vi "AlliGator Parameter Map Panel.vi"() -> ()   [LabVIEW 2021, in "AlliGator Parameter Map.lvlib"]
uses:
  AlliGator Parameter Map.lvlib
  AlliGator Parameter Map Control Refnums.ctl
  Globals, Variables, Constants/AlliGator Refnums List.ctl
  Utilities/Read-Write.ctl
  Settings/AlliGator Settings List.ctl
  Action Engine/AlliGator Q Element.ctl
  Action Engine/AlliGator Q Event.ctl
  Globals, Variables, Constants/AlliGator Variables List.ctl
  Palette/Image Palette Information.ctl
  Image/Image Display Palette Type.ctl
  Image/Image Display Event.ctl
  Image/Image Control Refnum.ctl
  <vilib>/Utility/miscctls.llb/LVPoint32TypeDef.ctl
  AlliGator Parameter Map Update Event Data.ctl
  GUI/AlliGator Image Mouse Up Event Data.ctl
  Image/Image ROI Descriptor.ctl
  Image/Image Contour Definition.ctl
  Image/Image Contour ID.ctl
  Image/Image ROI Type.ctl
  AlliGator Parameter Map Display Range Mouse Move Data.ctl
  Variant/Variant to Data/Variant to Boolean.vi
  Variant/Variant to Data/Variant to [String].vi
  Settings/AlliGator Settings+.lvlib
  Variant/Variant to Data/Variant to Data.lvlib
  Notebook/Notebook.lvlib
  Action Engine/AlliGator Action Engine.lvlib
  GUI/GUI.lvlib
  GUI/AlliGator GUI.lvlib
  Error/Error.lvlib
  Image/Image.lvlib
  Palette/Palette.lvlib
  Globals, Variables, Constants/AlliGator Globals, Variables & Constants.lvlib
  Python Plugins API/AlliGator Python Plugins.lvlib
  Phasor Plot/AlliGator Phasor Plot.lvlib
  Utilities/Utilities.lvlib
panel:
  in  "Map Parameter":u16(ring)
  in  "Parameter Map Set":u16(ring)
  in  "Pin Button":bool=TRUE
  in  "Overlay Parameter Map":bool caption="Overlay Decay Fit Parameter Map"
  in  "Parameter ROI Color":u32(colorbox)=6618880 caption="Phasor Plot ROI Color"
  in  "Refresh Parameter Map":bool caption="Refresh Phsor Plot"
  out "Parameter Map Display":T1(plugin-control)
  out "Parameter Map Value":dbl caption="Map Value" format="%#_5e"
  out "Parameter Map Y":i32 caption="Y"
  out "Parameter Map X":i32 caption="X"
  out "Min Parameter":dbl format="%#_5e"
  out "Max Parameter":dbl=1.0 format="%#_5e"
  in  "Parameter Map Color Scale":dbl(ramp)
  in  "Parameter Map Display Range":cluster{dbl, dbl}(slide)={0.0, 1.0} scale=9931.5..63525.26 scale format="%04_3g"
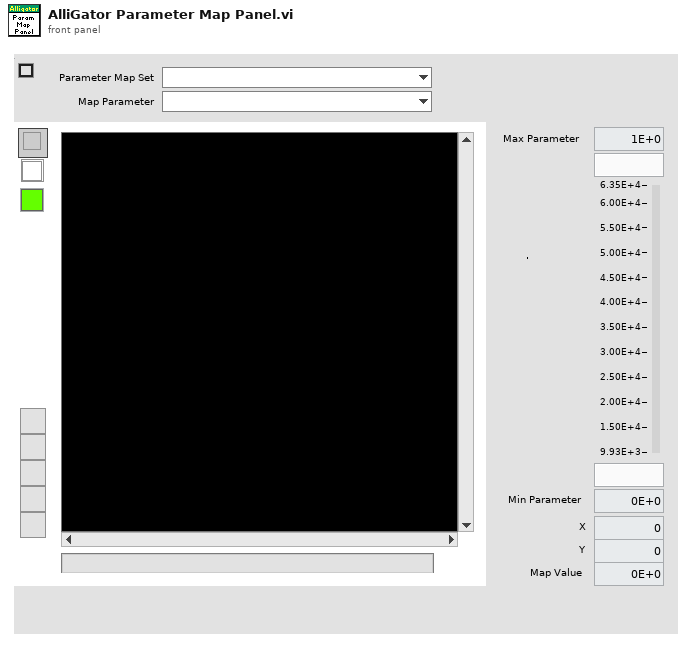
[diagram p1: front panel]
types:
  T1 = typedef "IMAQ Image.ctl" = refnum<image>
  T2 = typedef "Utilities.lvlib/Read-Write.ctl" = enum16{"Read", "Write"}
  T3 = typedef "AlliGator GUI.lvlib/AlliGator Refnums List.ctl" = enum16{"---------- AlliGator Control Refnums ----------", "AlliGator Tab Control Refnum", "Dataset Ctrl Refnums", "Image Histogram Ctrl Refnums", "Intensity Time Trace Ctrl Refnums", "Decay Graph Ctrl Refnums", "Decay Statistics Graph Ctrl Refnums", "Phasor Graph Ctrl Refnums", "Phasor Ratio Graph Ctrl Refnums", "Phasor Plot Ctrl Refnums", "Lifetime & Other Parameters Ctrl Refnums", "Decay Fit Parameter Map Ctrl Refnums", "Parameter Map Ctrl Refnums", "Other AlliGator Ctrl Refnums", "---------- AlliGator Menu Refnums ----------", "AlliGator Menu", "---------- IO Device ID ----------", "Mouse ID", "Keyboard ID"}
  T4 = typedef "AlliGator Parameter Map.lvlib/AlliGator Parameter Map Control Refnums.ctl" = cluster{"Parameter Map Color Scale":refnum<vi>, "Map Parameter":refnum<vi>, "Max Parameter":refnum<vi>, "Min Parameter":refnum<vi>, "Parameter Map Display":refnum<vi>, "Parameter Map Display Range":refnum<vi>, "Parameter Map Set":refnum<vi>, "Parameter Map X":refnum<vi>, "Parameter Map Y":refnum<vi>, "Parameter Map Value":refnum<vi>}
  T5 = cluster{"Event Registration Refnum":refnum<event-registration>, "Parameter Map Display Range Event":refnum<event-registration>, "Parameter Map Display Event":refnum<event-registration>}
  T6 = typedef "AlliGator Settings+.lvlib/AlliGator Settings List.ctl" = enum16{"GUI:Visible Settings Tab", "GUI:Last Run Version", "Source Image:Use Image Histogram for Contrast", "Source Image:Low Count Pixels Rejection Options", "Source Image:High Count Pixels Rejection Options", "Source Image:Use Image Brightness", "Source Image:Blend Overlay with Image Background", "Source Image:Use Fixed ROI Diameter", "Source Image:ROI Diameter", "Source Image:ROI Center Color", "Source Image:Peak Threshold", "Source Image:Intensity Threshold", "Source Image:Image Binning Options", "Source Image:Image Smoothing Options", "Source Image:Image Histogram Active", "Source Image:Invert Binary Mask", "Source Image:Hot Pixel Removal", "Source Image:Overlay Analyzed ROI Center", "Source Image:Auto-Adjust Contrast", "Source Image:Histogram Lower Percentile", "Source Image:Histogram Upper Percentile", "Source Image:Lock ROI with Maps", "Source Image:Save Source Image", "Source Image:Scale Bar Options", "Source Image:Image Resolution (Pixel Size)", "Source Image:Flatfield Correction", "Source Image:Show Dead Left Columns Correction", "Source Image:Dead Left Columns Correction", "Source Image:Image Pre-Processing Operations Order", "Source Image:Overlay ROI Median", "Source Image:Median Overlay Color", "Data Information:Gate Width", "Data Information:Nanotime Gate Separation", "Data Information:Macrotime Gate Separation", "Data Information:Gate Step", "Data Information:# Gates", "Data Information:Gate Image Exposure", "Data Information:Gate Image Integration", "Data Information:Gates to Skip", "Data Information:Gates to Keep", "Data Information:Define Gates to", "Data Information:Channel Name", "Data Information:Available Channel Names", "Data Information:Channel Arithmetic", "Data Information:Background File Subtraction", "Data Information:Background File", "Data Information:Background Scaling Factor", "Data Information:Background Pile-up Correction", "Data Information:Background Pixel Well Capacity", "Data Information:Laser Period", "Data Information:SYNC Period", "Data Information:Pile-up Correction", "Data Information:Pixel Well Capacity", "Data Information:Dataset Scaling Factor", "Fluorescence Decay_Decay Pre-Processing:Reverse Gates", "Fluorescence Decay_Decay Pre-Processing:Verbose Decay Pre-Processing", "Fluorescence Decay_Decay Pre-Processing:Use Decay Pre-Processing", "Fluorescence Decay_Decay Pre-Processing:Background Subtraction", "Fluorescence Decay_Decay Pre-Processing:Background Definition Range", "Fluorescence Decay_Decay Pre-Processing:Baseline Subtraction Method", "Fluorescence Decay_Decay Pre-Processing:Decay Pre-Processing Operations Order", "Fluorescence Decay_Decay Pre-Processing:Smoothing Parameter", "Fluorescence Decay_Decay Pre-Processing:Shift Decay", "Fluorescence Decay_Decay Pre-Processing:Decay Shift Parameters", "Fluorescence Decay_Decay Pre-Processing:Fold Decay", "Fluorescence Decay_Decay Pre-Processing:# Folds", "Fluorescence Decay_Decay Pre-Processing:1-Normalize Decay", "Fluorescence Decay_Decay Pre-Processing:[0-1]-Normalize Decay", "Fluorescence Decay_Decay Pre-Processing:Smoothen Decay", "Fluorescence Decay_Decay Pre-Processing:Extrapolate Decay", "Fluorescence Decay_Decay Pre-Processing:Use Periodicity", "Fluorescence Decay_Decay Pre-Processing:Use Cursors", "Fluorescence Decay_Decay Pre-Processing:Tail Fraction", "Fluorescence Decay_Decay Pre-Processing:Head Fraction", "Fluorescence Decay_Decay Pre-Processing:Additional Points", "Fluorescence Decay_Decay Pre-Processing:Straighten Decay", "Fluorescence Decay_Decay Pre-Processing:Constant Background", "Fluorescence Decay_Decay Pre-Processing:Pixel-Normalize Decay", "Fluorescence Decay_Advanced Analysis:Extract IRF instead of Decay", "Fluorescence Decay_Advanced Analysis:IRF Extraction Options", "Fluorescence Decay_Advanced Analysis:IRF Optimization Options", "Fluorescence Decay_Advanced Analysis:Square Pulse Options", "Fluorescence Decay_Advanced Analysis:IRF Order", "Fluorescence Decay_Advanced Analysis:IRF Time Constants", "Fluorescence Decay_Advanced Analysis:Wavelet Analysis Options", "Fluorescence Decay_Advanced Analysis:Average Lifetime Options", "Fluorescence Decay_Fit Options:Fit Options", "Fluorescence Decay_Fit Options:Use Legacy Fitting Approach", "Fluorescence Decay_Fit Options:Use Data Information Laser Period", "Fluorescence Decay_Fit Parameters:Displayed Fit Parameters", "Fluorescence Decay_Fit Parameters:Fit Parameter Constraints", "Fluorescence Decay_Fit Parameters:Export Tabulated Results", "Fluorescence Decay_Fit Parameters:MLE Baseline Offset Type", "Fluorescence Decay_Fit Parameters:MLE Baseline Offset", "Fluorescence Decay_Fit Parameters:Guess Parameter Names", "Fluorescence Decay_Fit Parameters:Guess Parameter Values", "Fluorescence Decay_Fit Parameters:Guess Parameters Options", "Fluorescence Decay_Fit Parameters:Optimal Offset Selection Criterion", "Fluorescence Decay_Styles:Show Last Decay Only", "Fluorescence Decay_Styles:Decay Graph Color Array", "Fluorescence Decay:Decay Graph Active", "Fluorescence Decay Statistics:Min Peak Value", "Fluorescence Decay Statistics:Reject Low Decay Peak Pixels", "Fluorescence Decay Statistics:Reject High Decay Peak Pixels", "Fluorescence Decay Statistics:Max Peak Value", "Time Traces:Use File Timestamp", "Time Traces:Time Step", "Time Traces:Use Intensity Correction File", "Time Traces:Intensity Correction File", "Phasor Plot:Phasor Plot Smoothing Options", "Phasor Plot:Phasor Plot Size", "Phasor Plot:Phasor Plot Graphics Options", "Phasor Plot:Cumulative Phasor Plot", "Phasor Plot:Use Phasor Brightness", "Phasor Plot:Blend Overlay with Phasor Background", "Phasor Plot:Save Phasor Plot", "Phasor Plot:Show References", "Phasor Plot:Phasor Ratio Decay Range", "Phasor Plot:Exponential Fading", "Phasor Plot:Phasor Ratio Reference Colors", "Phasor Plot:Reference Radius", "Phasor Plot:Show Color Map Vertices", "Phasor Plot:Phasor Plot Active", "Phasor Plot:Phasor Ratio Color Map Type", "Phasor Plot:Phasor Ratio Color Map", "Phasor Plot:Phasor Ratio Display Range", "Phasor Plot:Selected Image ROI(s)", "Phasor Plot:All Image ROIs", "Phasor Plot:Selected Phasor Plot ROI(s)", "Phasor Plot:All Phasor Plot ROIs", "Phasor Plot:Phasor Ratio Color-Coded Quantity", "Phasor Plot:Store Phasor Harmonics", "Phasor Plot:Draw Reference Segment", "Phasor Plot:User-Defined Quantity", "Phasor Plot:Color Scale High Color", "Phasor Plot:Color Scale Low Color", "Phasor Plot:Intensity-weighted Phasor Plot", "Phasor Graph:Phasor Frequency", "Phasor Graph:Phasor Ratio Type", "Phasor Graph:Pixel-level Phasor Computation", "Phasor Graph:Save Phasor Graph", "Phasor Graph:Phasor Graph Active", "Phasor Graph:Phasor SDV Options", "Phasor Graph:Intensity-weighted Phasor Graph", "Phasor Graph:Define Shortest Lifetime as", "Phasor Calibration:Use Backup Calibration if needed", "Phasor Calibration:Backup Calibration Type", "Phasor Calibration:Calibration Type", "Phasor Calibration:Calibration Lifetime", "Phasor Calibration:Calibration Map Algorithm", "Single-Exponential Phasor Locus (SEPL):Gate Parameters", "Single-Exponential Phasor Locus (SEPL):User-defined Gate", "Single-Exponential Phasor Locus (SEPL):User-defined IRF", "Single-Exponential Phasor Locus (SEPL):Phasor Parameters", "Single-Exponential Phasor Locus (SEPL):Decay & IRF Parameters", "Single-Exponential Phasor Locus (SEPL):Display Parameters", "Lifetime Analysis:Decay Analysis Parameters", "Lifetime Analysis:Lifetime Map Active", "Plugins:Python Settings", "Miscellaneous:Verbose Mode", "Miscellaneous:Beep after Script", "Miscellaneous:Saved Image File Format", "Miscellaneous:Exported Gate Image Settings", "Miscellaneous:Include Loading in Timing", "Miscellaneous:Verbose Settings Mode", "Miscellaneous:Histogram Options", "Miscellaneous:Beep on Error", "Miscellaneous:# Logical Processors Used", "Miscellaneous:ROI Description Max Characters", "Miscellaneous:Verbose Error Mode", "Miscellaneous:Transparent Mask Color"}
  T7 = typedef "AlliGator Action Engine.lvlib/AlliGator Q Element.ctl" = cluster{"AlliGator Q Event":T8, "Data":variant}
  T8 = typedef "AlliGator Action Engine.lvlib/AlliGator Q Event.ctl" = enum16{"---- Files ----", "Files:Set Batch Export Files To Save", "Files:Set Dataset Loading & Pre-processing Options", "Files:Check #Frames in Dataset", "Files:Increment Frame Index", "Files:Open Mask Image", "Files:Open White Light Image", "Files:Open Single Dataset", "Files:New Folder of Folders Selected", "Files:Load File (all Types)_Scriptable", "Files:Move Flattened Series to Folders Series", "Files:Select Folder", "Files:Load FLI Dataset", "Files:Load Swiss SPAD 1 Dataset", "Files:Load Swiss SPAD 2 Dataset", "Files:Load .sdt FLI Dataset", "Files:Load .ptu FLI Dataset", "Files:Load .bin FLI Dataset", "Files:Load Single Gate Image Folder", "Files:Load I/m/phi Dataset (deprecated)", "Files:Load Single Image", "Files:Subtract Background File", "Files:Export FLI Dataset", "Files:Load HDF5 FLI Dataset", "Files:Set Destination File Path", "Files:Save Mask Image", "Files:Batch Conversion", "Files:New Folder Selected", "Files:Close FLI Dataset", "Files:Close FLI Dataset Series", "Files:Close White Light Image", "Files:Close Mask Image", "---- FLI Dataset ----", "FLI Dataset:Channel Arithmetic", "FLI Dataset:Export Average Lifetime Map as ASCII", "FLI Dataset:Export User-Defined Quantity Map as ASCII", "FLI Dataset:Python Function FLI Dataset Event", "FLI Dataset:ROI Analysis", "FLI Dataset:Tilted Logistic Square Gated IRF Characteristics Map", "FLI Dataset:Logistic Square Gated IRF Characteristics Map", "FLI Dataset:Square Gated IRF Characteristics Map", "FLI Dataset:Multi-ROI Single-Pixel Phasor Analysis", "FLI Dataset:Multi-ROI Single-Pixel NLSF Analysis", "FLI Dataset:All ROIs IRF Extraction", "FLI Dataset:All ROIs Decay Fit Non-Interactive (Fast + Individual IRF)", "FLI Dataset:All ROIs Phasor Analysis", "FLI Dataset:All ROIs Decay Fit", "FLI Dataset:Fluorescence Decay Statistics", "FLI Dataset:Update Decay Statistics Graph", "FLI Dataset:Get Decay from ROI", "FLI Dataset:All ROIs Average Lifetimes", "FLI Dataset:Save/Load Local IRFs", "FLI Dataset:Clear Local IRFs", "FLI Dataset:Phasor Calibration Maps (# Gates Series) Script", "FLI Dataset:Calibrated Phasor Map Series", "---- FLI Dataset Series ----", "FLI Dataset Series:Sum All Datasets in Series", "FLI Dataset Series:Add Dataset to Accumulated Dataset", "FLI Dataset Series:Display Accumulated Dataset", "FLI Dataset Series:Clear Dataset Series Sum", "FLI Dataset Series:Time-Series Analysis (NLSF)", "FLI Dataset Series:Time-Series Analysis (Phasor)", "---- Image ----", "Image:Update Image Profile Plots", "Image:Image Histogram Cursor Move", "Image:Image Histogram", "Image:Image Contrast", "Image:Set Image Histogram Cursor Move Flag", "Image:Clear Image Overlay", "Image:Use ROI as Search Area", "Image:Set ROI Diameter", "Image:Save Image Data as TIFF", "Image:Save Displayed Image with Overlay", "Image:Save Image Overlay Only", "Image:Save Image as Hot Pixel Mask", "Image:Change Source Image Color Palette", "Image:Copy Image to Clipboard", "Image:Source Image ROI Selection", "Image:Delete All ROIs", "Image:Delete All Unselected ROIs", "Image:Delete ROI", "Image:Merge All ROIs", "Image:Store ROI", "Image:Source Image ROI Storage", "Image:Export ROI Description to Notebook", "Image:Save ROI", "Image:Load ROI", "Image:Paste ROI Definition", "Image:Clear ROI", "Image:Identify ROIs in Mask Image", "Image:Create Complementary ROI", "Image:Create Contour ROI", "Image:Create ROI(s) from Pixels with Peak above Min_Scriptable", "Image:Create ROI(s) from Pixels with Intensity above Min_Scriptable", "Image:Compute ROI Statistics", "Image:Delete ROI(s) based on ROI Characteristics", "Image:Create ROI Grid", "Image:ROI to Individual Pixel ROIs", "Image:Python Function Source Image Event", "Image:Show Phasor Calibration Map ROI Centers", "Image:Convert ROI to Mask Image", "Image:Mouse Move", "Image:Mouse Up", "Image:Set Source Image Mouse Move Flag", "Image:Add Scale Bar Overlay", "Image:Delete Existing ROIs Option", "Image:Overlay ROI Median", "Image:Check Current ROI", "Image:Update True Pixel Value", "Image:Use ROI", "---- Decay ----", "Decay:Clear IRF/Reference Plot", "Decay:Add Decay to Graph", "Decay:Smoothen Plot", "Decay:Smoothen Plot Tail", "Decay:Average Selected Plots", "Decay:Extract IRF", "Decay:Optimal IRF Extraction", "Decay:Threshold IRF", "Decay:Fit to Model IRF", "Decay:Fit IRF to Square Gate", "Decay:Fit IRF to Logistic Square Gate", "Decay:Fit IRF to Tilted Logistic Square Gate", "Decay:Create Bounding Cursors Set", "Decay:Export Bounding Cursors Definition to Notebook", "Decay:Denoise Plot", "Decay:Compute Cumulative Function", "Decay:Use as Reference Decay", "Decay:Show Reference Decay/IRF", "Decay:Extrapolate Decay", "Decay:Create Head & Tail Bounding Cursors", "Decay:Store Cursor-defined Head & Tail Fractions", "Decay:Rebin Plot", "Decay:1-Normalize Decay", "Decay:[0-1]-Normalize Plot", "Decay:Straighten Decay", "Decay:Shift Decay", "Decay:Fold Decay", "Decay:Fit Decay", "Decay:Global Fit of Selected Decays", "Decay:Post Global Fit Script", "Decay:Add Global Fit Parameters to Graph", "Decay:Add Decay Parameter(s) to Plot (Graph)", "Decay:Export Decay to Phasor Graph", "Decay:Compute Average Lifetime", "Decay:Plot Convolution", "Decay:Graph Tip Strip Update", "---- Decay Statistics ----", "Decay Statistics:Tip Strip Update", "---- Intensity Time Trace ----", "Intensity Time Trace:Use File Timestamp", "Intensity Time Trace:Load Intensity Corrections File", "Intensity Time Trace:Clear Intensity Corrections File", "Intensity Time Trace:Tip Strip Update", "---- Phasor Plot ----", "Phasor Plot:Build Phasor Plot", "Phasor Plot:Change Phasor Plot Color Palette", "Phasor Plot:Adjust Phasor Plot Display Range", "Phasor Plot:Highlight Image ROI in Phasor Plot", "Phasor Plot:Save Phasor Plot Image with Overlay", "Phasor Plot:Export Complex Phasor Map", "Phasor Plot:Export Phasor Ratio Map", "Phasor Plot:Export Average Lifetime Map", "Phasor Plot:Compute Phase Lifetime Histogram", "Phasor Plot:Compute Phasor Ratio Histogram", "Phasor Plot:Compute Phase Lifetime vs Intensity Scatter Plot", "Phasor Plot:Weber 2-Component Decomposition", "Phasor Plot:Update Phasor Color Map Vertices", "Phasor Plot:Clear Phasor Overlay", "Phasor Plot:Use Segment Extremities as References", "Phasor Plot:Use UC/Segment Intersections as References", "Phasor Plot:Use UC/Principal Axis Intersections as References", "Phasor Plot:Use UC/Linear Fit Intersections as References", "Phasor Plot:Update Phasor Plot Reference", "Phasor Plot:Show Local Phasor Info in Phasor Plot", "Phasor Plot:Update Phasor Plot State", "Phasor Plot:Phasor Plot ROI Storage", "Phasor Plot:Phasor Plot ROI Selection", "Phasor Plot:Python Function Phasor Plot Event", "Phasor Plot:Overlay Phasor ROI, Ratio or Map in Source Image", "Phasor Plot:Compute Decay of Selected Phasors", "Phasor Plot:Phasor at Image Pixel", "Phasor Plot:Mouse Move", "Phasor Plot:Mouse Up", "Phasor Plot:Display Range Mouse Move", "Phasor Plot:Set Mouse Move Flag", "Phasor Plot:Update True Phasor Plot Value", "---- Phasor Graph ----", "Phasor Graph:Get Phasor Value", "Phasor Graph:Create New Phasor Plot Dialog", "Phasor Graph:Update Last Phasor Value", "Phasor Graph:Update Phasor (m, phi)", "Phasor Graph:Remove Single Phasor from Plot", "Phasor Graph:Add Single Phasor to Plot", "Phasor Graph:Remove Phasor Plot", "Phasor Graph:Remove Selected Phasor Plots", "Phasor Graph:Clear Phasor Data", "Phasor Graph:Clear Phasor Graph", "Phasor Graph:Cursor Move", "Phasor Graph:Draw Cursor Connecting Line", "Phasor Graph:Clear Cursor Connecting Line", "Phasor Graph:Find UC Intersection", "Phasor Graph:Use UC/Cursor-Defined Line Intersections", "Phasor Graph:Use Selected Plots Fitted Line/UC Intersections", "Phasor Graph:Use Selected Plots Principal Axis/UC Intersections", "Phasor Graph:Show Single Phasor", "Phasor Graph:Save Single Phasor Plot", "Phasor Graph:Save All Phasor Plots", "Phasor Graph:Load Phasor Plot(s)", "Phasor Graph:Phasor Multiplication", "Phasor Graph:Compute Average Phasor", "Phasor Graph:Compute Multiple Average Phasors (Selected Plots)", "Phasor Graph:Export Single Phasor Plot Phase Lifetimes", "Phasor Graph:Parameter 2 vs Parameter 1 Scatter Plot", "Phasor Graph:Use Cursor n Location", "Phasor Graph:Set Reference n to Current Phase Lifetime Value", "Phasor Graph:Set Reference n to Lifetime Value", "Phasor Graph:Set Cursor n Location", "Phasor Graph:Save Phasor Graph Image", "Phasor Graph:Update SEPL Plot", "Phasor Graph:Export Single Phasor Plot Data", "Phasor Graph:Export Selected Phasor Plots Data", "Phasor Graph:Python Function Phasor Graph Event", "Phasor Graph:Tip Strip Update", "---- Calibration ----", "Calibration:Set Calibration Type", "Calibration:Load/Save Phasor Calibration", "Calibration:Load/Save Phasor Calibration Series", "Calibration:Load/Save Phasor Calibration Map", "Calibration:Use as Calibration", "Calibration:Compute Optimal Calibration from Phasor References", "Calibration:Clear Phasor Calibration", "Calibration:Single Phasor Calibration Information", "Calibration:Use as Calibration Series", "Calibration:Use as Calibration Map", "Calibration:Clear Calibration Series", "Calibration:Phasor Calibration Series Information", "Calibration:Clear Calibration Map", "Calibration:Phasor Calibration Map Information", "Calibration:Apply Phasor Calibration", "Calibration:Update Single Plot Calibration", "Calibration:Update Multiple Plots Calibration", "Calibration:Clear Single Plot Calibration", "Calibration:Clear All Plots Calibrations", "Calibration:Clear Plot(s) Calibration(s)?", "---- Phasor Ratio ----", "Phasor Ratio:Clear Reference n", "Phasor Ratio:Toggle Selected Plot(s)  Lock to Reference 1", "Phasor Ratio:Use as Reference n", "Phasor Ratio:Send Reference n to Notebook", "Phasor Ratio:Toggle Selected Plot(s)  Lock to Reference 2", "Phasor Ratio:Compute Phasor Ratio at Mouse Location", "Phasor Ratio:Compute Phasor Plot's Average Phasor Ratio", "Phasor Ratio:Compute Time-Series Phasor Ratios", "Phasor Ratio:Fit Line to Phasor Ratio Plot", "Phasor Ratio:Save References", "Phasor Ratio:Load References", "Phasor Ratio:Update Phasor Reference 1", "Phasor Ratio:Update Phasor Reference 2", "Phasor Ratio:Move Cursor n to Reference n", "Phasor Ratio:Use as Phasor Reference 1 Lifetime", "Phasor Ratio:Use as Phasor Reference 2 Lifetime", "Phasor Ratio:Export Phasor Ratio Map as ASCII", "Phasor Ratio:Tip Strip Update", "---- Lifetime & Other Parameters Graph ----", "Lifetime:Compute Sliced Mean, SDV and CV Plots", "Lifetime:Plot Decay Shifts", "Lifetime:Plot Histogram", "---- Decay Fit Parameter Map ----", "Decay Fit Parameter Map:Export ROI NLSF Data as ASCII", "Decay Fit Parameter Map:Set Decay Fit Parameter Map Selection", "Decay Fit Parameter Map:Build Decay Fit Parameter Map", "Decay Fit Parameter Map:Change Decay Fit Parameter Map Color Palette", "Decay Fit Parameter Map:Export Decay Fit Parameter Map Data as ASCII", "Decay Fit Parameter Map:Export All Decay Fit Parameter Maps Data as ASCII", "Decay Fit Parameter Map:Selected Parameter Scatterplot", "Decay Fit Parameter Map:Parameter 2 vs Parameter 1 Scatterplot", "Decay Fit Parameter Map:Save Decay Fit Parameter Map Image", "Decay Fit Parameter Map:Save-Load IRFs & Fit Data", "Decay Fit Parameter Map:Update Local Decay Plots", "Decay Fit Parameter Map:Python Function Decay Fit Parameters Map Event", "Decay Fit Parameter Map:Overlay Decay Fit Parameter Map in Source Image", "Decay Fit Parameter Map:Selected Parameter vs Intensity Scatterplot", "Decay Fit Parameter Map:Mouse Up", "Decay Fit Parameter Map:Mouse Move", "Decay Fit Parameter Map:Display Range Mouse Move", "Decay Fit Parameter Map:Change Map Resolution", "Decay Fit Parameter Map:Variance Significance Maps", "Decay Fit Parameter Map:Fit Result Constraints Window", "Decay Fit Parameter Map:Use ROI", "---- Parameter Map ----", "Parameter Map:Export ROI Parameters Data as ASCII", "Parameter Map:Add Parameter Map Set", "Parameter Map:Delete Parameter Map Set", "Parameter Map:Update Parameter List", "Parameter Map:Build Parameter Map", "Parameter Map:Change Parameter Map Color Palette", "Parameter Map:Export Parameter Map Data as ASCII", "Parameter Map:Export All Parameter Maps Data as ASCII", "Parameter Map:Selected Parameter Scatterplot", "Parameter Map:Parameter 2 vs Parameter 1 Scatterplot", "Parameter Map:Selected Parameter vs Intensity Scatterplot", "Parameter Map:Save Parameter Map Image", "Parameter Map:Save-Load IRFs & Parameter Maps (TODO)", "Parameter Map:Set Parameter Map Selection", "Parameter Map:Python Function Parameter Map Event", "Parameter Map:Overlay Parameter Map in Source Image", "Parameter Map:Update Local Decay Plots", "Parameter Map:Mouse Up", "Parameter Map:Mouse Move", "Parameter Map:Display Range Mouse Move", "Parameter Map:Use ROI", "---- Generic Graph ----", "Generic Graph:Generic XY Graph Event", "Generic Graph:Python Function XY Graph Event", "Generic Graph:New Plot", "Generic Graph:Save Plot", "Generic Graph:XY Plot Histogram", "Generic Graph:Set XY Graph Plot Name", "Generic Graph:Set Last Cursor Style", "Generic Graph:Tip Strip Update", "---- GUI ----", "GUI:Start Script", "GUI:Type of Displayed Image Changed", "GUI:Gate Image Slide Changed", "GUI:Show Busy Icon", "GUI:Show Busy Icon & Abort Button", "GUI:Hide Busy Icon", "GUI:Hide Busy Icon & Abort Button", "GUI:Abort", "GUI:End Script", "GUI:Start Timing", "GUI:End Timing", "GUI:Set State Indicator", "GUI:Send Parameters JSON Strings to Clipboard", "GUI:Set Gate Step", "GUI:Idle", "GUI:Initialization", "GUI:Quit", "GUI:Increment Dataset Index", "GUI:Set Dataset Index to -1", "GUI:Time Series Slider Moved", "GUI:Time Series Slider Changed", "GUI:Toggle Playback or Loop", "GUI:Playback Script", "GUI:Set Phasor Frequency", "GUI:Open Window", "GUI:Start Test Script", "GUI:End Test Script", "GUI:Set Verbose Mode", "GUI:Set Verbose Settings Mode", "GUI:Initialize Python Session", "DEBUG"}
  T9 = typedef "Palette.lvlib/Image Palette Information.ctl" = cluster{"Palette Name [# Colors,int?,inv?]":string, "Palette Type":T10, "Palette Colors":u32[], "Interpolate?":bool}
  T10 = typedef "Image.lvlib/Image Display Palette Type.ctl" = u32
  T11 = typedef "AlliGator Globals, Variables & Constants.lvlib/AlliGator Variables List.ctl" = enum16{"---- GUI ----", "GUI:Initialization Status", "GUI:State Indicators Refnum", "GUI:Original AlliGator Menu Items", "GUI:Current Action Loop State", "GUI:Script in progress", "GUI:Playback", "GUI:Loop Playback", "GUI:Search ROI Used", "GUI:Search ROI", "Image Histogram Max Legend Size", "Decay Graph Max Legend Size", "Intensity Graph Max Legend Size", "Decay Statistics Graph Max Legend Size", "Phasor Graph Max Legend Size", "Phasor Ratio Graph Max Legend Size", "Lifetime Graph Max Legend Size", "---- Files ----", "Files:Export Dataset Frames as Individual Files", "Files:Show Batch Export Help Balloons", "Files:Frames in Dataset", "Files:ptu File Frame Start Indices", "Files:Current Frame in Dataset", "Files:Current Frame Timestamp", "Files:Dataset Loaded", "Files:Dataset Metadata", "Files:Dataset Channel", "Files:Dataset Data Description", "Files:Background Dataset Metadata", "Files:Background Dataset Channel", "Files:Background Dataset Data Description", "Files:Background File Subtraction", "Files:Background File Path", "Files:Background File Pile-up Correction", "Files:Background File Pixel Well Capacity", "Files:Background File Scaling Factor", "Files:Current Dataset Load Settings", "Files:Dataset Path", "Files:ICCD-specific Information", "Files:Macrotime Gate Separation", "------ Python Plugins ------", "Python Plugins:Information", "Python Plugins:Python Session", "Python Plugins:Valid Python Session?", "---- Source Image ----", "Source Image:ROIs", "Source Image:Current ROI", "Source Image:ROI Event Refnum", "X_Source Image:Display Range", "X_Source Image:Palette Information", "X_Source Image:Type of Displayed Image", "X_Time Gate Slider", "Source Image:Palette List", "Source Image:Scale", "Source Image:ROI Overlay Color", "Source Image:Overlay to Erase", "Source Image:Is Displayed Image Accumulated", "Source Image:White Light Image Modified", "Source Image:Mask Image Modified", "---- Image Profile Window ----", "Image Profile:Window Event Refnum", "Image Profile:IntensityType", "Image Profile:Intensity Average Type", "Image Profile:Intensity-weighted SDV", "Image Profile:Box Profile Type", "Image Profile:Window Open", "Image Profile:Plotted Fit Parameter", "------ Phasor Graph -------", "Phasor Graph:Show Line", "---- Phasor Plot ---", "Phasor Plot:Parameters Changed", "Phasor Plot:FLI Dataset Modified since last Calculation", "Phasor Harmonics Data", "Selected Phasor Harmonics", "Phasor Harmonic Manager Event Refnum", "Phasor Plot:ROIs", "Phasor Plot:Current ROI", "Phasor Plot:ROI Event Refnum", "Phasor Plot:Image Reference Points", "Phasor Plot:Computed", "Phasor Plot:Palette Information", "Phasor Plot:Palette List", "Phasor Plot:Phasor Ratio Palette Information", "Phasor Plot:Phasor Ratio Palette List", "Phasor Plot:Image Scale", "Phasor Plot:Image Overlay to Erase", "Phasor Plot:Image Elements to Update", "Phasor Plot:Current Calculation Parameters", "Phasor Plot:Current Calibration Options", "Phasor Plot:Reset Cumulated Phasor Plot", "Phasor Plot:Reference 1", "Phasor Plot:Lifetime Reference 1", "Phasor Plot:Reference 1 Frequency", "Phasor Plot:Reference 2", "Phasor Plot:Lifetime Reference 2", "Phasor Plot:Reference 2 Frequency", "---- Decay Analysis ----", "Number of Selected Decays to Fit", "LS Fit Results", "LAR Fit Results", "BS Fit Results", "Last Decay Max - Min", "Best Fit Parameters", "Best Fit Parameter Names", "Actual Size X", "Actual Size Y", "Binning X", "Binning Y", "Actual # Gates", "Dataset Number", "Gates to...", "Gates Skipped", "Gates to keep", "Gate Step", "Gate Separation", "Reversed Gates", "Pile-up Correction", "Pixel Well Capacity", "Background Subtracted", "Background Subtraction Method", "Background Definition Range", "Background File (deprecated)", "Number of Dataset Accumulated", "Array of Accumulated Dataset Paths", "Do Averaged Datasets", "Destination File Path", "Process Plot Target", "Use 1/D as Phasor Frequency", "---- Decay Fit Parameter Map -----", "Decay Fit Parameter Map:Palette Information", "Decay Fit Parameter Map:Palette List", "Decay Fit Parameter Map:X Resolution", "Decay Fit Parameter Map:Y Resolution", "Decay Fit Parameter Map:Use Decay Fit Result Constraints", "Decay Fit Parameter Map:Decay Fit Result Constraints", "Decay Fit Parameter Map:Decay Fit Result Constraints Applied", "---- Parameter Map ----", "Parameter Map:Palette Information", "Parameter Map:Palette List", "------- Local Decay Window ---------", "Local Decay Graph Window:Event Refnum", "Local Decay Graph Window:Use normalized IRF for convolution", "----- Miscellaneous ----", "Misc:Skippable Dialog Windows Status"}
  T12 = enum16{"0", "1", "2", "3", "4", "5", "6", "7", "8", "9", "A", "B", "C", "D", "E", "F", "G", "H", "I", "J", "K", "L", "M", "N", "O", "P", "Q", "R", "S", "T", "U", "V", "W", "X", "Y", "Z", "F1", "F2", "F3", "F4", "F5", "F6", "F7", "F8", "F9", "F10", "F11", "F12", "F13", "F14", "F15", "ADD", "BACK", "BACKSLASH", "CAPITAL", "COMMA", "DECIMAL", "DELETE", "DIVIDE", "DOWN", "END", "EQUALS", "ESCAPE", "GRAVE (`)", "HOME", "INSERT", "LBRACKET", "LCONTROL", "LEFT", "L ALT", "LSHIFT", "LWIN", "MINUS", "MULTIPLY", "NEXT", "NUMLOCK", "NUMPAD_0", "NUMPAD_1", "NUMPAD_2", "NUMPAD_3", "NUMPAD_4", "NUMPAD_5", "NUMPAD_6", "NUMPAD_7", "NUMPAD_8", "NUMPAD_9", "PAUSE", "PERIOD", "PRIOR (PG UP)", "RBRACKET", "RCONTROL", "RETURN", "RIGHT", "R ALT", "RSHIFT", "RWIN", "SCROLL", "SEMICOLON", "SLASH", "SPACE", "SUBTRACT", "TAB", "UP", "ENTER (num pad)", "' (quote)"}
  T13 = typedef "Image.lvlib/Image Display Event.ctl" = cluster{"Item Tag":string, "Image Control Refnum":T14, "Coords":T15, "Item Path":string}
  T14 = typedef "Image.lvlib/Image Control Refnum.ctl" = refnum<vi>
  T15 = typedef "LVPoint32TypeDef.ctl" = cluster{"Horizontal":i32, "Vertical":i32}
  T16 = typedef "AlliGator Parameter Map.lvlib/AlliGator Parameter Map Update Event Data.ctl" = cluster{"Parameter":u16, "Parameter changed":bool, "Map Set":u16}
  T17 = typedef "AlliGator GUI.lvlib/AlliGator Image Mouse Up Event Data.ctl" = cluster{"Current ROI Tool":u32, "ROI Descriptor":T18, "Shift":bool, "Alt":bool, "Image Display Refnum":T14}
  T18 = typedef "Image.lvlib/Image ROI Descriptor.ctl" = cluster{"Global Rectangle":i32[], "Contours":T19[]}
  T19 = typedef "Image.lvlib/Image Contour Definition.ctl" = cluster{"Contour Type":T20, "ROI Type":T21, "Points":i32[]}
  T20 = typedef "Image.lvlib/Image Contour ID.ctl" = enum32{"External", "Internal"}
  T21 = typedef "Image.lvlib/Image ROI Type.ctl" = enum16{"No Selection", "Point", "Line", "Rectangle", "Oval", "Polygon", "Freehand Region", "Annulus", "Unused2", "Unused3", "Broken Line", "Freehand Line", "Rotated Rectangle"}
  T22 = typedef "AlliGator Parameter Map.lvlib/AlliGator Parameter Map Display Range Mouse Move Data.ctl" = cluster{"Parameter Map Set":u16, "Map Parameter":u16}
  T23 = enum16{"0", "1", "2", "3", "4", "5", "6", "7", "8", "9", "A", "B", "C", "D", "E", "F", "G", "H", "I", "J", "K", "L", "M", "N", "O", "P", "Q", "R", "S", "T", "U", "V", "W", "X", "Y", "Z", "F1", "F2", "F3", "F4", "F5", "F6", "F7", "F8", "F9", "F10", "F11", "F12", "F13", "F14", "F15", "ADD", "BACK", "BACKSLASH", "CAPITAL", "COMMA", "DECIMAL", "DELETE", "DIVIDE", "DOWN", "END", "EQUALS", "ESCAPE", "GRAVE (`)", "HOME", "INSERT", "LBRACKET", "LCONTROL", "LEFT", "L ALT", "LSHIFT", "LWIN", "MINUS", "MULTIPLY", "NEXT", "NUMLOCK", "NUMPAD_0", "NUMPAD_1", "NUMPAD_2", "NUMPAD_3", "NUMPAD_4", "NUMPAD_5", "NUMPAD_6", "NUMPAD_7", "NUMPAD_8", "NUMPAD_9", "PAUSE", "PERIOD", "PRIOR (PG UP)", "RBRACKET", "RCONTROL", "RETURN", "RIGHT", "R ALT", "RSHIFT", "RWIN", "SCROLL", "SEMICOLON", "SLASH", "SPACE", "SUBTRACT", "TAB", "UP", "ENTER (num pad)", "' (quote)"}[]
  T24 = cluster{"button 1":bool, "button 2":bool, "button 3":bool, "button 4":bool}
  T25 = cluster{"Global Rectangle":i32[], "Contours":cluster{"Contour Type":u32, "ROI Type":u32, "Points":i32[]}[]}
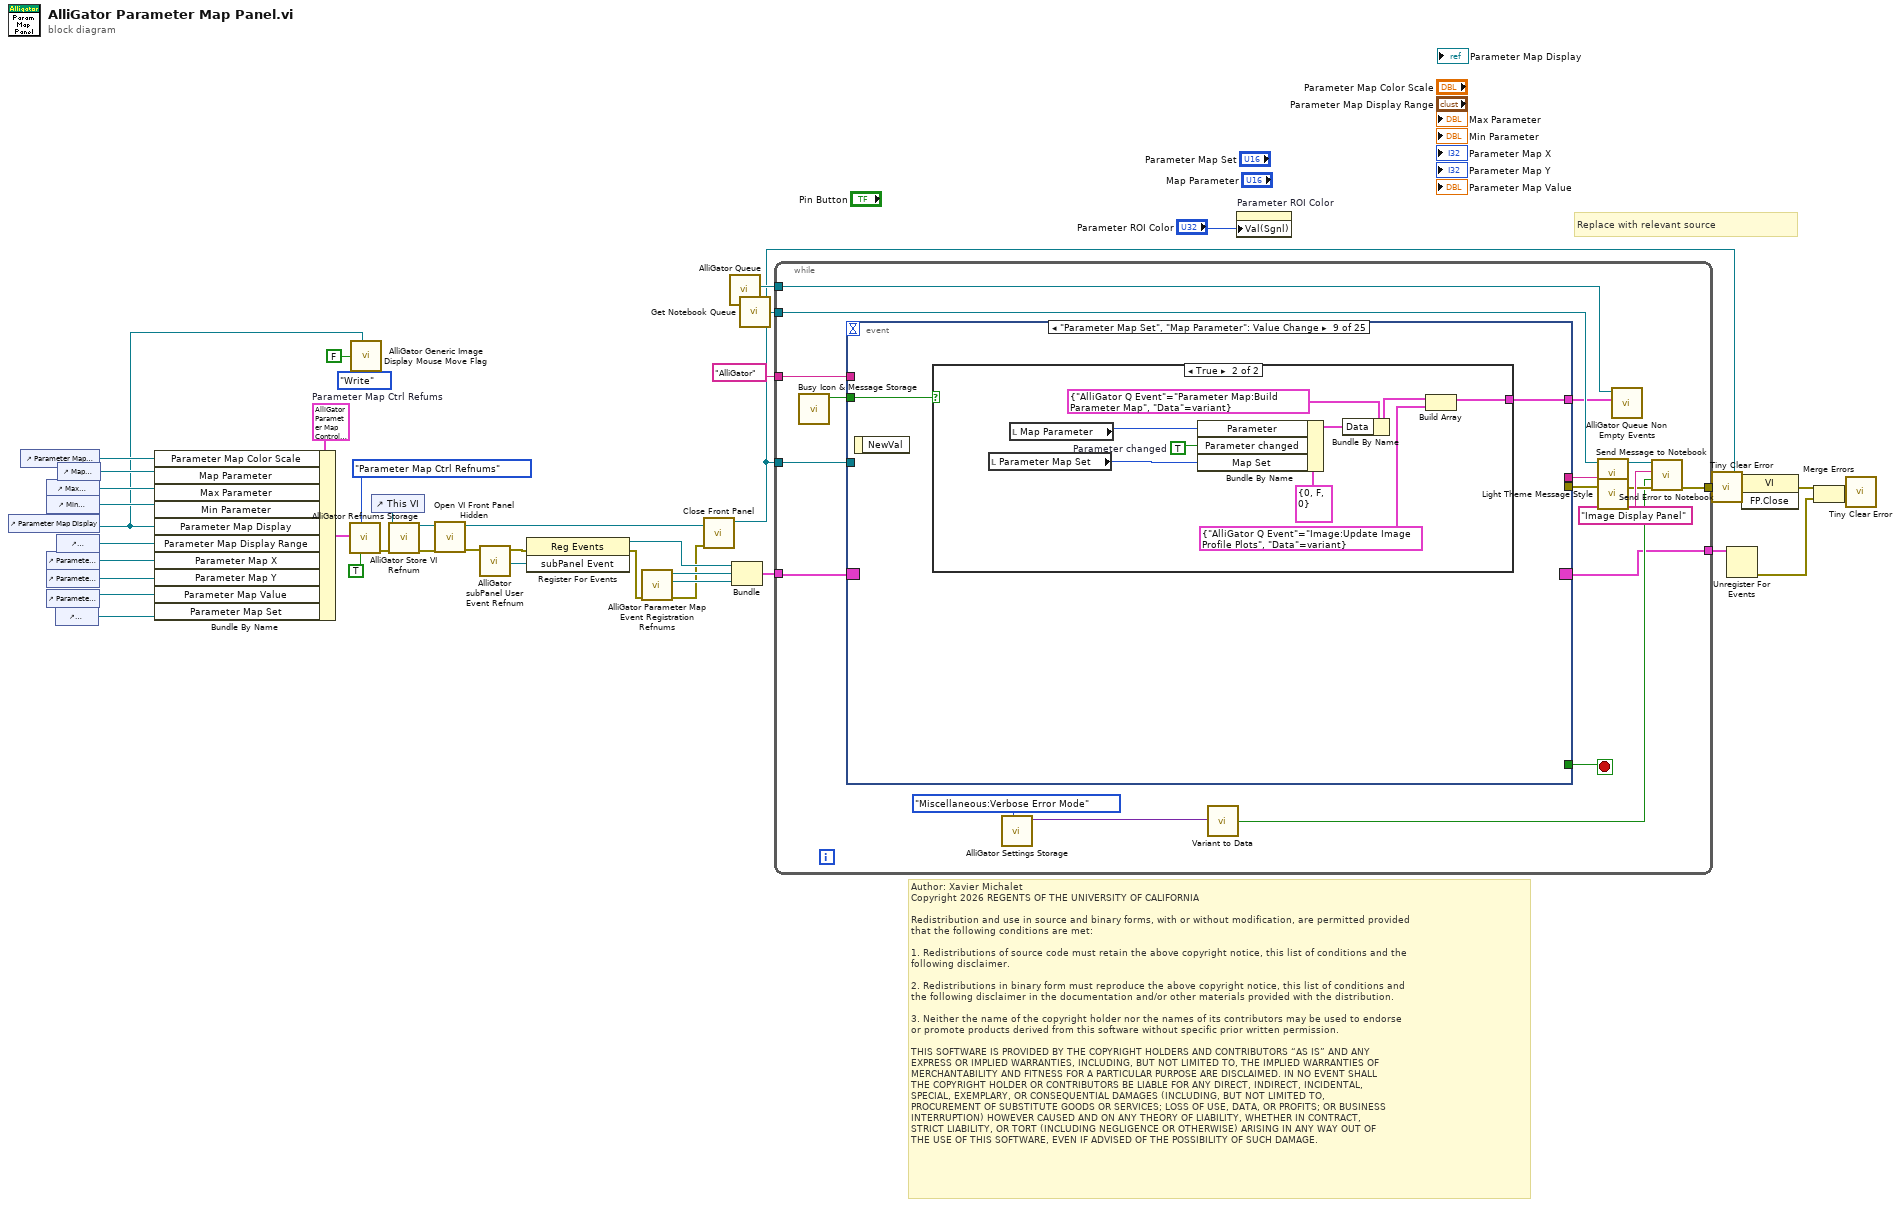
[diagram p0: block diagram]
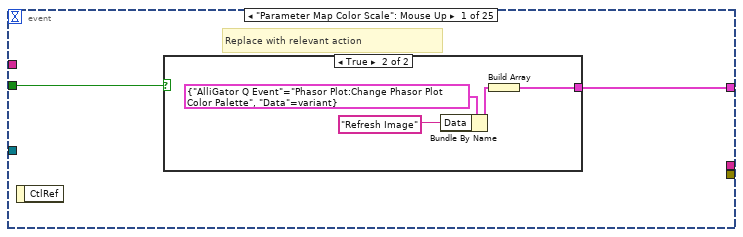
[diagram p2: hidden frame]
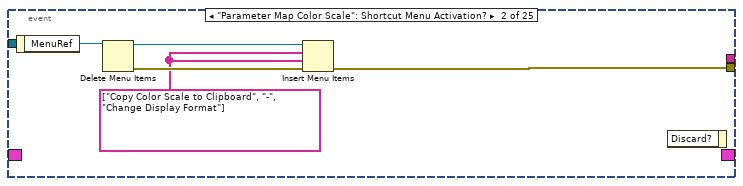
[diagram p4: hidden frame]
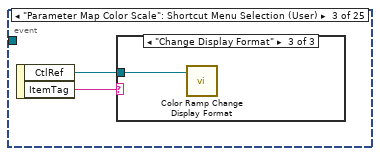
[diagram p5: hidden frame]
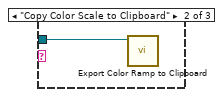
[diagram p7: hidden frame]
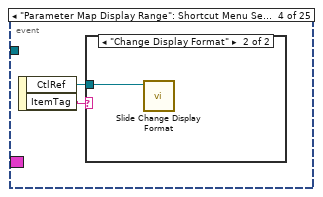
[diagram p8: hidden frame]
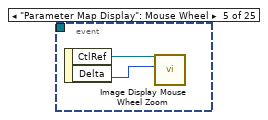
[diagram p10: hidden frame]
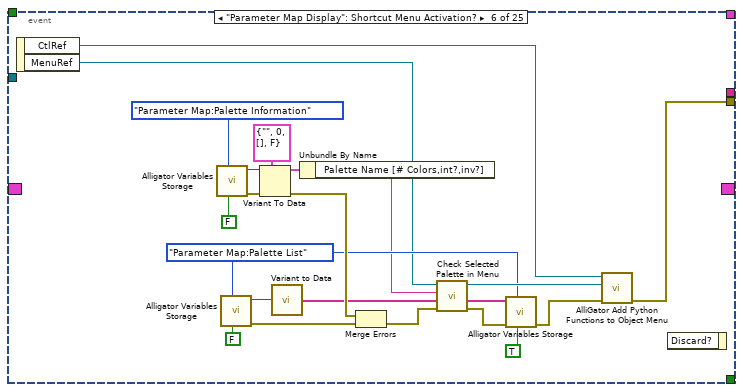
[diagram p11: hidden frame]
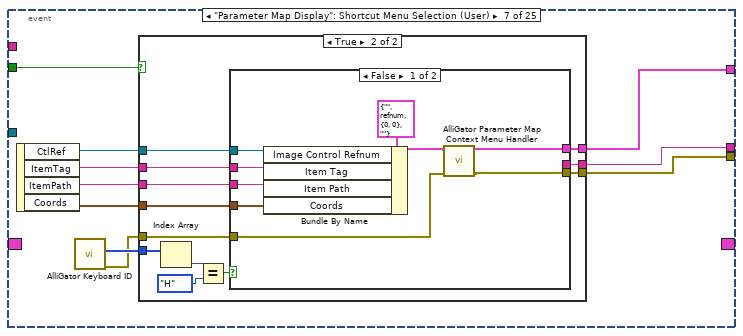
[diagram p12: hidden frame]
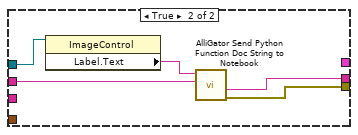
[diagram p14: hidden frame]
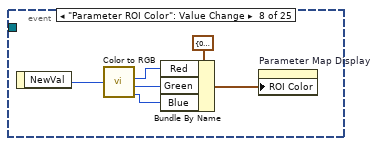
[diagram p15: hidden frame]
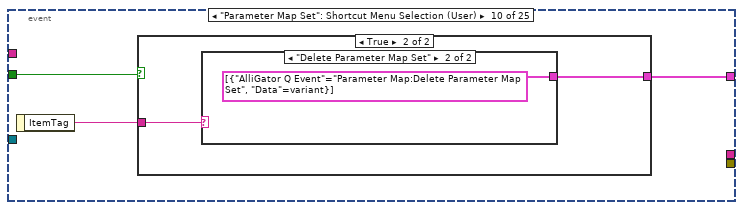
[diagram p17: hidden frame]
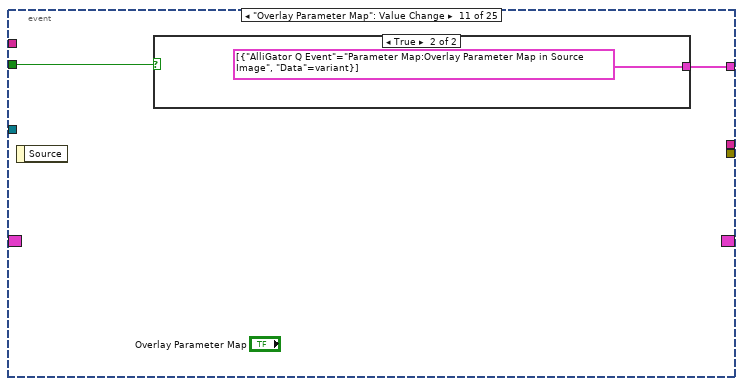
[diagram p20: hidden frame]
diagram:
  w24 = T4 {"Parameter Map Color Scale"=refnum, "Map Parameter"=refnum, "Max Parameter"=refnum, "Min Parameter"=refnum, "Parameter Map Display"=refnum, "Parameter Map Display Range"=refnum, "Parameter Map Set"=refnum, "Parameter Map X"=refnum, "Parameter Map Y"=refnum, "Parameter Map Value"=refnum}  # Parameter Map Ctrl Refums
  # "Replace with relevant source"
  # "Author: Xavier Michalet\nCopyright 2026 REGENTS OF THE UNIVERSITY OF CALIFORNIA\n\nRedistribution and use in source and binary forms, with or without modification, are permitted provided\nthat the following conditions are met:\n\n1. Redistributions of source code must retain the above copyright notice, this list of conditions and the\nfollowing disclaimer.\n\n2. Redistributions in binary form must reproduce the above copyright notice, this list of conditions and\nthe following disclaimer in the documentation and/or other materials provided with the distribution.\n\n3. Neither the name of the copyright holder nor the names of its contributors may be used to endorse \nor promote products derived from this software without specific prior written permission.\n\nTHIS SOFTWARE IS PROVIDED BY THE COPYRIGHT HOLDERS AND CONTRIBUTORS “AS IS” AND ANY \nEXPRESS OR IMPLIED WARRANTIES, INCLUDING, BUT NOT LIMITED TO, THE IMPLIED WARRANTIES OF\nMERCHANTABILITY AND FITNESS FOR A PARTICULAR PURPOSE ARE DISCLAIMED. IN NO EVENT SHALL\nTHE COPYRIGHT HOLDER OR CONTRIBUTORS BE LIABLE FOR ANY DIRECT, INDIRECT, INCIDENTAL, \nSPECIAL, EXEMPLARY, OR CONSEQUENTIAL DAMAGES (INCLUDING, BUT NOT LIMITED TO, \nPROCUREMENT OF SUBSTITUTE GOODS OR SERVICES; LOSS OF USE, DATA, OR PROFITS; OR BUSINESS\nINTERRUPTION) HOWEVER CAUSED AND ON ANY THEORY OF LIABILITY, WHETHER IN CONTRACT, \nSTRICT LIABILITY, OR TORT (INCLUDING NEGLIGENCE OR OTHERWISE) ARISING IN ANY WAY OUT OF\nTHE USE OF THIS SOFTWARE, EVEN IF ADVISED OF THE POSSIBILITY OF SUCH DAMAGE."
  n1 = control-ref of="Parameter Map Display"() -> (w5:refnum<vi>)
  n2 = control-ref of="Parameter Map Color Scale"() -> (w23:refnum<vi>)
  n3 = control-ref of="Max Parameter"() -> (w17:refnum<vi>)
  n4 = control-ref of="Min Parameter"() -> (w21:refnum<vi>)
  n5 = control-ref of="Parameter Map X"() -> (w20:refnum<vi>)
  n6 = control-ref of="Parameter Map Y"() -> (w19:refnum<vi>)
  n7 = control-ref of="Parameter Map Value"() -> (w18:refnum<vi>)
  n8 = control-ref of="Parameter Map Set"() -> (w13:refnum<vi>)
  n9 = control-ref of="Parameter Map Display Range"() -> (w22:refnum<vi>)
  n10 = control-ref of="Map Parameter"() -> (w14:refnum<vi>)
  n11 = Bundle By Name(cluster=w24, "Parameter Map Color Scale"=w23, "Map Parameter"=w14, "Max Parameter"=w17, "Min Parameter"=w21, "Parameter Map Display"=w5, "Parameter Map Display Range"=w22, "Parameter Map X"=w20, "Parameter Map Y"=w19, "Parameter Map Value"=w18, "Parameter Map Set"=w13) -> (w25:T4)
  n12 = call "AlliGator Refnums Storage.vi"("Get(F)/Set"=TRUE, "AlliGator Refnum List"=AlliGator_Refnums_List."Parameter Map Ctrl Refnums", "Data in"=w25) -> ("Error Out"=w4:errorcluster)  [unwired: 7 in, 1 out]
  n13 = call "AlliGator Generic Image Display Mouse Move Flag.vi"("Image Control Refnum"=w5, "Flag (in)"=FALSE, "Read/Write"=Read-Write."Write") -> ()  [unwired: 6 in, 1 out]
  n14 = control-ref of="This VI"() -> (w2:refnum<vi>)
  n15 = call "AlliGator Store VI Refnum.vi"("error in (no error)"=w4, "VI Refnum"=w2) -> ("error out"=w3:errorcluster, "VI Refnum (dup)"=w1:refnum<vi>)  [unwired: 7 in, 1 out]
  n16 = call "Open VI Front Panel Hidden.vi"("error in"=w3, "VI in"=w1) -> ("error out"=w12:errorcluster, "VI out"=w10:refnum<vi>)  [unwired: 8 in]
  n17 = call "AlliGator subPanel User Event Refnum.vi"() -> ("subPanel Event"=w37:refnum<user-event>)  [unwired: 9 in]
  n18 = register-events(error in=w12, w37) -> (reference out=w36:refnum<event-registration>, error out=w11:errorcluster)  [unwired: 1 in]
  n19 = call "AlliGator Parameter Map Event Registration Refnums.vi"("error in (no error)"=w11) -> ("error out"=w9:errorcluster, "Parameter Map Display Event"=w15:refnum<event-registration>, "Parameter Map Display Range Event"=w16:refnum<event-registration>)  [unwired: 8 in]
  n20 = call "Close Front Panel.vi"("error in (no error)"=w9, "VI in"=w10) -> ("VI out"=w8:refnum<vi>)  [unwired: 8 in, 1 out]
  n21 = call "AlliGator Queue.vi"() -> ("AlliGator Q"=w39:refnum<queue>)  [unwired: 8 in, 1 out]
  n22 = Bundle("Event Registration Refnum"=w36, "Parameter Map Display Range Event"=w16, "Parameter Map Display Event"=w15) -> (w32:T5)  [unwired: 1 in]
  n23 = call "Get Notebook Queue.vi"() -> ("Notebook Queue"=w40:refnum<queue>)  [unwired: 9 in]
  n24 = while {
    tunnel: w40 -> [w51]
    tunnel: w39 -> [w48]
    tunnel: "AlliGator" ("Sender") -> [w46]
    tunnel: w8 -> [w44]
    tunnel: w32 -> [w41]
    tunnel: [w43] -> w35
    tunnel: [w42] -> w34
    stop <- w58 stop-if-true
    n25 = call "Busy Icon & Message Storage.vi"() -> ("Busy Icon Status (F = busy)"=w45:bool)  [unwired: 9 in, 2 out]
    n26 = event shown="[8] \"Parameter Map Set\", \"Map Parameter\": Value Change" {
      selector: w41 -> [_ _ _ _ _ _ _ _ _ _ _ _ _ _ _ w185 w198 _ w225 w248 _ w268 w274 _ _]
      dyn-events: [_ _ _ _ _ _ _ _ _ _ _ _ _ _ _ w184 w196 _ w224 w247 _ w269 w275 _ _] -> w43
      timeout: _ -> [_ _ _ _ _ _ _ _ _ _ _ _ _ _ _ _ _ _ _ _ _ _ _ _ _]
      tunnel: [_ w65 _ _ _ w79 w103 _ _ _ _ w163 w166 w168 _ w181 w194 _ _ _ _ _ _ _ w300] -> w52
      tunnel: [_ _ _ _ _ _ _ _ _ _ _ _ _ _ _ _ _ _ _ _ _ _ _ w292 _] -> w58
      tunnel: [_ _ _ _ _ _ w104 _ _ _ _ _ _ _ _ _ _ _ _ _ _ _ _ _ _] -> w49
      tunnel: [w60 _ _ _ _ _ w105 _ w143 w156 w161 _ _ _ w172 _ _ w211 w227 _ w253 _ w279 _ _] -> w47
      tunnel: w45 -> [w59 _ _ _ _ _ w106 _ w144 w154 w160 _ _ _ w171 w182 w195 w209 w226 _ w252 _ w278 _ _]
      tunnel: w46 -> [_ _ _ _ _ _ _ _ _ _ _ _ _ _ _ _ _ _ _ _ _ _ _ _ _]
      tunnel: w44 -> [_ _ _ _ _ _ _ _ _ _ _ w165 _ _ _ _ _ _ _ _ _ _ _ _ w299]
      event "Parameter Map Color Scale": Mouse Up {
        # "Replace with relevant action"
        n27 = event-data() -> ()  [unwired: 1 in, 1 out]
        n28 = case shown="True" w59 {
          tunnel: [_ w61] -> w60
          frame False {
          }
          frame True {
            n29 = Bundle By Name(cluster=T7 {"AlliGator Q Event"=enum."Phasor Plot:Change Phasor Plot Color Palette", "Data"=variant} ("element"), "Data"="Refresh Image" ("String")) -> (w63:T7)
            n30 = Build Array(w63) -> (w61:T7[])
          }
        }
      }
      event "Parameter Map Color Scale": Shortcut Menu Activation? {
        w68 = string[] ["Copy Color Scale to Clipboard", "-", "Change Display Format"] ("item names")
        n31 = event-data() -> ("MenuRef"=w66:refnum<k9>)  [unwired: 1 in]
        n32 = Delete Menu Items(9:w66) -> (0:w69:errorcluster, 3:w67:refnum<k9>)  [unwired: 3 in]
        n33 = Insert Menu Items(6:w69, 7:w68, 8:w68, 9:w67) -> (0:w65:errorcluster)  [unwired: 2 in, 2 out]
        n34 = event-data() -> ()  [unwired: 2 in, 1 out]
      }
      event "Parameter Map Color Scale": Shortcut Menu Selection (User) {
        n35 = event-data() -> ("CtlRef"=w71:refnum<vi>, "ItemTag"=w70:string)  [unwired: 1 in]
        n36 = case shown="\"Change Display Format\"" w70 {
          tunnel: w71 -> [_ w72 w73]
          frame "", Default {
          }
          frame "Copy Color Scale to Clipboard" {
            n37 = call "Export Color Ramp to Clipboard.vi"("ColorRamp Refnum"=w72) -> ()  [unwired: 11 in]
          }
          frame "Change Display Format" {
            n38 = call "Color Ramp Change Display Format.vi"("ColorRamp Refnum"=w73) -> ()  [unwired: 10 in, 1 out]
          }
        }
      }
      event "Parameter Map Display Range": Shortcut Menu Selection (User) {
        n39 = event-data() -> ("CtlRef"=w75:refnum<vi>, "ItemTag"=w74:string)  [unwired: 1 in]
        n40 = case shown="\"Change Display Format\"" w74 {
          tunnel: w75 -> [_ w76]
          frame "", Default {
          }
          frame "Change Display Format" {
            n41 = call "Slide Change Display Format.vi"("Slide Refnum"=w76) -> ()  [unwired: 10 in, 1 out]
          }
        }
      }
      event "Parameter Map Display": Mouse Wheel {
        n42 = event-data() -> ("CtlRef"=w78:refnum<vi>, "Delta"=w77:i32)  [unwired: 1 in]
        n43 = call "Image Display Mouse Wheel Zoom.vi"("Mouse Wheel Delta"=w77, "Image Control Refnum"=w78) -> ()  [unwired: 9 in, 1 out]
      }
      event "Parameter Map Display": Shortcut Menu Activation? {
        w94 = AlliGator_Variables_List."Parameter Map:Palette List" ("Alligator Variable")
        n44 = event-data() -> ("CtlRef"=w80:refnum<vi>, "MenuRef"=w81:refnum<k9>)  [unwired: 1 in]
        n45 = call "Alligator Variables Storage.vi"("Get(F)/Set"=FALSE, "AlliGator Variable"=AlliGator_Variables_List."Parameter Map:Palette Information" ("Alligator Variable")) -> ("Error Out"=w85:errorcluster, "Data out"=w84:variant)  [unwired: 7 in, 1 out]
        n46 = call "Alligator Variables Storage.vi"("Get(F)/Set"=FALSE, "AlliGator Variable"=w94) -> ("Error Out"=w97:errorcluster, "Data out"=w90:variant)  [unwired: 7 in, 1 out]
        n47 = Variant To Data(error in=w85, type=T9 {"Palette Name [# Colors,int?,inv?]"="", "Palette Type"=0, "Palette Colors"=[], "Interpolate?"=FALSE} ("Image Display Palette Information"), Variant=w84) -> (data=w86:T9, error out=w95:errorcluster)
        n48 = call-poly "Variant to Data.vi"("Variant"=w90) -> ("String Array"=w91:string[])  [unwired: 8 in]
        n49 = Unbundle By Name(w86) -> ("Palette Name [# Colors,int?,inv?]"=w88:string)
        n50 = Merge Errors(w95, w97) -> (w96:errorcluster)
        n51 = call "Check Selected Palette in Menu.vi"("Error In"=w96, "Palette List"=w91, "Checked Palette"=w88, "Menu in"=w81) -> ("Error Out"=w98:errorcluster, "Stored Palette List"=w93:string[], "menu reference out"=w99:refnum<k9>)  [unwired: 5 in]
        n52 = call "Alligator Variables Storage.vi"("Get(F)/Set"=TRUE, "AlliGator Variable"=w94, "Error In"=w98, "Data in"=w93) -> ("Error Out"=w100:errorcluster)  [unwired: 5 in, 2 out]
        n53 = call "AlliGator Add Python Functions to Object Menu.vi"("error in (no error)"=w100, "Menu in"=w99, "Object Refnum"=w80) -> ("error out"=w79:errorcluster)  [unwired: 6 in, 2 out]
        n54 = event-data() -> ()  [unwired: 2 in, 1 out]
      }
      event "Parameter Map Display": Shortcut Menu Selection (User) {
        n55 = event-data() -> ("CtlRef"=w110:refnum<vi>, "ItemTag"=w109:string, "ItemPath"=w108:string, "Coords"=w107:T15)  [unwired: 1 in]
        n56 = call "AlliGator Keyboard ID.vi"() -> ("error out"=w101:errorcluster, "keys pressed"=w102:T23)  [unwired: 9 in, 1 out]
        n57 = case shown="True" w106 {
          tunnel: w110 -> [_ w122]
          tunnel: w108 -> [_ w121]
          tunnel: w109 -> [_ w120]
          tunnel: [_ w119] -> w105
          tunnel: w107 -> [_ w118]
          tunnel: w102 -> [_ w114]
          tunnel: [_ w113] -> w104
          tunnel: [_ w112] -> w103
          tunnel: w101 -> [_ w111]
          frame False {
          }
          frame True {
            n58 = Index Array(array=w114) -> (element=w117:T12)  [unwired: 1 in]
            n59 = Equal?(x=w117, y=T12."H" ("element")) -> (x = y?=w115:bool)
            n60 = case shown="False" w115 {
              tunnel: w122 -> [w130 w135]
              tunnel: w121 -> [w128 _]
              tunnel: w120 -> [w129 w134]
              tunnel: [w125 _] -> w119
              tunnel: w118 -> [w127 _]
              tunnel: [_ w133] -> w113
              tunnel: [w124 w132] -> w112
              tunnel: w111 -> [w123 _]
              frame False {
                n61 = Bundle By Name(cluster=T13 {"Item Tag"="", "Image Control Refnum"=refnum, "Coords"={"Horizontal"=0, "Vertical"=0}, "Item Path"=""} ("Image Event Data"), "Image Control Refnum"=w130, "Item Tag"=w129, "Item Path"=w128, "Coords"=w127) -> (w126:T13)
                n62 = call "AlliGator Parameter Map Context Menu Handler.vi"("Error In"=w123, "Image Event Data"=w126) -> ("Error Out"=w124:errorcluster, "AlliGator Actions"=w125:T7[])  [unwired: 8 in]
              }
              frame True {
                n63 = property class="ImageControl"(reference=w135) -> ("Label.Text"=w136:string)  [unwired: 1 in, 2 out]
                n64 = call "AlliGator Send Python Function Doc String to Notebook.vi"("Item Tag"=w134, "Target"=w136) -> ("Error Out"=w132:errorcluster, "Message"=w133:string)  [unwired: 8 in]
              }
            }
          }
        }
      }
      event "Parameter ROI Color": Value Change {
        n65 = event-data() -> ("NewVal"=w138:u32)  [unwired: 1 in]
        n66 = call <vilib>:"Color to RGB.vi"("Color"=w138) -> ("R"=w141:u8, "G"=w140:u8, "B"=w139:u8)  [unwired: 1 out]
        n67 = Bundle By Name(cluster=cluster{"Red":u8, "Green":u8, "Blue":u8} {"Red"=0, "Green"=0, "Blue"=0} ("ROI Color"), "Red"=w141, "Green"=w140, "Blue"=w139) -> (w137:cluster{"Red":u8, "Green":u8, "Blue":u8})
        n68 = property on="Parameter Map Display" class="ImageControl"("ROI Color"=w137) -> ()  [unwired: 2 in, 2 out]
      }
      event "Parameter Map Set", "Map Parameter": Value Change {
        n69 = event-data() -> ()  [unwired: 1 in, 1 out]
        n70 = case shown="True" w144 {
          tunnel: [_ w148] -> w143
          frame False {
          }
          frame True {
            w149 = TRUE  # Parameter changed
            n71 = local read "Parameter Map Set"() -> (w146:u16)
            n72 = local read "Map Parameter"() -> (w145:u16)
            n73 = Bundle By Name(cluster=T16 {"Parameter"=0, "Parameter changed"=FALSE, "Map Set"=0} ("output cluster"), "Parameter"=w145, "Parameter changed"=w149, "Map Set"=w146) -> (w150:T16)
            n74 = Bundle By Name(cluster=T7 {"AlliGator Q Event"=enum."Parameter Map:Build Parameter Map", "Data"=variant} ("Time-Gated Phasor Q Element"), "Data"=w150) -> (w152:T7)
            n75 = Build Array(w152, T7 {"AlliGator Q Event"=enum."Image:Update Image Profile Plots", "Data"=variant} ("Time-Gated Phasor Q Element")) -> (w148:T7[])
          }
        }
      }
      event "Parameter Map Set": Shortcut Menu Selection (User) {
        n76 = event-data() -> ("ItemTag"=w155:string)  [unwired: 1 in]
        n77 = case shown="True" w154 {
          tunnel: w155 -> [_ w158]
          tunnel: [_ w157] -> w156
          frame False {
          }
          frame True {
            n78 = case shown="\"Delete Parameter Map Set\"" w158 {
              tunnel: [_ T7[] [{"AlliGator Q Event"=enum."Parameter Map:Delete Parameter Map Set", "Data"=variant}] ("AlliGator Actions")] -> w157
              frame "", Default {
              }
              frame "Delete Parameter Map Set" {
              }
            }
          }
        }
      }
      event "Overlay Parameter Map": Value Change {
        n79 = event-data() -> ()  [unwired: 1 in, 1 out]
        n80 = case shown="True" w160 {
          tunnel: [_ T7[] [{"AlliGator Q Event"=enum."Parameter Map:Overlay Parameter Map in Source Image", "Data"=variant}] ("element")] -> w161
          frame False {
          }
          frame True {
          }
        }
      }
      event "Pin Button": Value Change {
        n81 = event-data() -> ("NewVal"=w164:bool)  [unwired: 1 in]
        n82 = call "AlliGator Dock-Undock Subpanel Event.vi"("Dock?"=w164, "VI in"=w165) -> ("Error Out"=w163:errorcluster)  [unwired: 9 in]
      }
      event "Refresh Parameter Map": Shortcut Menu Activation? {
        n83 = event-data() -> ("MenuRef"=w167:refnum<k9>)  [unwired: 1 in]
        n84 = call "AlliGator Set Checks in Phasor Update Button.vi"("Menu in"=w167) -> ("Error Out"=w166:errorcluster)  [unwired: 10 in]
        n85 = event-data() -> ()  [unwired: 2 in, 1 out]
      }
      event "Refresh Parameter Map": Shortcut Menu Selection (User) {
        n86 = event-data() -> ("ItemTag"=w170:string, "CtlRef"=w169:refnum<vi>)  [unwired: 1 in]
        n87 = call "AlliGator Update Phasor Image Elements to Update.vi"("CtlRef"=w169, "Phasor Plot Element to Update"=w170) -> ("Error Out"=w168:errorcluster)  [unwired: 8 in, 1 out]
      }
      event "Refresh Parameter Map": Value Change {
        n88 = event-data() -> ()  [unwired: 1 in, 1 out]
        n89 = case shown="True" w171 {
          tunnel: [_ w176] -> w172
          frame False {
          }
          frame True {
            w177 = TRUE  # Parameter changed
            n90 = local read "Parameter Map Set"() -> (w174:u16)
            n91 = local read "Map Parameter"() -> (w173:u16)
            n92 = Bundle By Name(cluster=T16 {"Parameter"=0, "Parameter changed"=FALSE, "Map Set"=0} ("output cluster"), "Parameter"=w173, "Parameter changed"=w177, "Map Set"=w174) -> (w178:T16)
            n93 = Bundle By Name(cluster=T7 {"AlliGator Q Event"=enum."Parameter Map:Build Parameter Map", "Data"=variant} ("Time-Gated Phasor Q Element"), "Data"=w178) -> (w179:T7)
            n94 = Build Array(w179) -> (w176:T7[])
          }
        }
      }
      event Mouse Enter {
        n95 = event-data() -> ("CtlRef"=w183:refnum<vi>)  [unwired: 1 in]
        n96 = case "Mouse Enter" shown="True" w182 {
          tunnel: [w186 w191] -> w184
          tunnel: w185 -> [w186 w190]
          tunnel: w183 -> [_ w187]
          tunnel: [_ w188] -> w181
          frame False {
          }
          frame True {
            n97 = Unbundle By Name(w190) -> ("Parameter Map Display Event"=w192:refnum<event-registration>)
            n98 = register-events(reference=w192, T14 refnum ("event source"), w187, w187, w187) -> (reference out=w193:refnum<event-registration>, error out=w188:errorcluster)  [unwired: 1 in]
            n99 = Bundle By Name(cluster=w190, "Parameter Map Display Event"=w193) -> (w191:T5)
          }
        }
      }
      event Mouse Leave {
        n100 = event-data() -> ("CtlRef"=w197:refnum<vi>)  [unwired: 1 in]
        n101 = case shown="True" w195 {
          tunnel: [w199 w204] -> w196
          tunnel: w198 -> [w199 w203]
          tunnel: w197 -> [_ w202]
          tunnel: [_ w201] -> w194
          frame False {
          }
          frame True {
            w200 = refnum<vi> refnum ("event source")
            n102 = Unbundle By Name(w203) -> ("Parameter Map Display Event"=w205:refnum<event-registration>)
            n103 = register-events(reference=w205, w202, w200, w200, w200) -> (reference out=w206:refnum<event-registration>, error out=w201:errorcluster)  [unwired: 1 in]
            n104 = Bundle By Name(cluster=w203, "Parameter Map Display Event"=w206) -> (w204:T5)
          }
        }
      }
      event Mouse Move {
        # "not busy and left button up"
        n105 = event-data() -> ("Time"=w213:u32, "CtlRef"=w212:refnum<vi>)  [unwired: 1 in]
        n106 = call "AlliGator Mouse ID.vi"() -> ("button info"=w210:T24)  [unwired: 8 in, 3 out]
        n107 = Unbundle By Name(w210) -> ("button 1"=w207:bool)
        n108 = Compound Arithmetic op=AND(w209, invert w207) -> (w208:bool)
        n109 = case shown="True" w208 {
          tunnel: w212 -> [_ w218]
          tunnel: [_ w214] -> w211
          tunnel: w213 -> [_ w220]
          frame False {
            # "if busy or the left button is down, do nothing"
          }
          frame True {
            w221 = T7 {"AlliGator Q Event"=enum."Parameter Map:Mouse Move", "Data"=variant} ("Array")
            n110 = call "AlliGator Filter Event.vi"("Time"=w220, "AlliGatorr Q Element"=w221) -> ("Filter Event?"=w217:bool)  [unwired: 8 in, 1 out]
            n111 = call "AlliGator Generic Image Display Mouse Move Flag.vi"("Image Control Refnum"=w218, "Read/Write"=Read-Write."Read") -> ("Flag (out)"=w216:bool)  [unwired: 7 in]
            n112 = Or(x=w217, y=w216) -> (x .or. y?=w215:bool)
            n113 = case shown="True" w215 {
              tunnel: w221 -> [w222 _]
              tunnel: w218 -> [_ _]
              tunnel: [w223 _] -> w214
              frame False {
                # "update X,Y,Value"
                n114 = Build Array(w222) -> (w223:T7[])
              }
              frame True {
                # "if not timed out AND action still unfolding, ignore event"
              }
            }
          }
        }
      }
      event Mouse Up {
        n115 = event-data() -> ("CtlRef"=w229:refnum<vi>, "PlatMods.Alt"=w228:bool)  [unwired: 1 in]
        n116 = case shown="True" w226 {
          tunnel: w229 -> [_ w235]
          tunnel: [_ w243] -> w227
          tunnel: w228 -> [_ w237]
          tunnel: w225 -> [w230 w233]
          tunnel: [w230 w231] -> w224
          frame False {
          }
          frame True {
            w234 = refnum<vi> refnum ("event source")
            n117 = property class="ImageControl"(reference=w235) -> (reference out=w242:refnum<vi>, "ROI"=w241:T25, "Current ROI Tool"=w240:u32)  [unwired: 1 in, 1 out]
            n118 = Unbundle By Name(w233) -> ("Parameter Map Display Event"=w236:refnum<event-registration>)
            n119 = Bundle By Name(cluster=T17 {"Current ROI Tool"=8, "ROI Descriptor"={"Global Rectangle"=[], "Contours"=[]}, "Shift"=FALSE, "Alt"=FALSE, "Image Display Refnum"=refnum} ("Phasor Plot Mouse Up Event Data"), "Image Display Refnum"=w242, "ROI Descriptor"=w241, "Current ROI Tool"=w240, "Alt"=w237) -> (w238:T17)
            n120 = register-events(reference=w236, w234, w234, w235, w235) -> (reference out=w232:refnum<event-registration>)  [unwired: 1 in, 1 out]
            n121 = Bundle By Name(cluster=w233, "Parameter Map Display Event"=w232) -> (w231:T5)
            n122 = Bundle By Name(cluster=T7 {"AlliGator Q Event"=enum."Parameter Map:Mouse Up", "Data"=variant} ("Array"), "Data"=w238) -> (w244:T7)
            n123 = Build Array(w244) -> (w243:T7[])
          }
        }
      }
      event Mouse Down {
        w251 = refnum<vi> refnum  # Slide (strict)
        n124 = event-data() -> ("CtlRef"=w246:refnum<vi>)  [unwired: 1 in]
        n125 = Unbundle By Name(w248) -> ("Parameter Map Display Range Event"=w250:refnum<event-registration>)
        n126 = register-events(reference=w250, w251, w246, w246, w246) -> (reference out=w249:refnum<event-registration>)  [unwired: 1 in, 1 out]
        n127 = Bundle By Name(cluster=w248, "Parameter Map Display Range Event"=w249) -> (w247:T5)
      }
      event Mouse Move {
        n128 = event-data() -> ("Time"=w254:u32)  [unwired: 1 in]
        n129 = case shown="True" w252 {
          tunnel: [_ w258] -> w253
          tunnel: w254 -> [_ w257]
          frame False {
          }
          frame True {
            w256 = T7 {"AlliGator Q Event"=enum."Parameter Map:Display Range Mouse Move", "Data"=variant} ("Time-Gated Phasor Q Element")
            n130 = call "AlliGator Filter Event.vi"("Time"=w257, "AlliGatorr Q Element"=w256) -> ("Filter Event?"=w255:bool)  [unwired: 8 in, 1 out]
            n131 = case shown="False" w255 {
              tunnel: [w264 _] -> w258
              tunnel: w256 -> [w263 _]
              frame False {
                n132 = local read "Parameter Map Set"() -> (w260:u16)
                n133 = local read "Map Parameter"() -> (w259:u16)
                n134 = Bundle(cluster=T22 {"Parameter Map Set"=0, "Map Parameter"=0}, "Parameter Map Set"=w260, "Map Parameter"=w259) -> (w261:T22)
                n135 = Bundle By Name(cluster=w263, "Data"=w261) -> (w265:T7)
                n136 = Build Array(w265) -> (w264:T7[])
              }
              frame True {
              }
            }
          }
        }
      }
      event Mouse Leave {
        w266 = refnum<vi> refnum  # Slide (strict)
        n137 = event-data() -> ("CtlRef"=w267:refnum<vi>)  [unwired: 1 in]
        n138 = Unbundle By Name(w268) -> ("Parameter Map Display Range Event"=w271:refnum<event-registration>)
        n139 = register-events(reference=w271, w267, w266, w266, w266) -> (reference out=w270:refnum<event-registration>)  [unwired: 1 in, 1 out]
        n140 = Bundle By Name(cluster=w268, "Parameter Map Display Range Event"=w270) -> (w269:T5)
      }
      event Mouse Up {
        w272 = refnum<vi> refnum  # Slide (strict)
        n141 = event-data() -> ("Time"=w280:u32, "CtlRef"=w273:refnum<vi>)  [unwired: 1 in]
        n142 = case shown="True" w278 {
          tunnel: [_ w284] -> w279
          tunnel: w280 -> [_ w283]
          frame False {
          }
          frame True {
            w282 = T7 {"AlliGator Q Event"=enum."Parameter Map:Display Range Mouse Move", "Data"=variant} ("Time-Gated Phasor Q Element")
            n143 = call "AlliGator Filter Event.vi"("Time"=w283, "AlliGatorr Q Element"=w282) -> ("Filter Event?"=w281:bool)  [unwired: 8 in, 1 out]
            n144 = case shown="False" w281 {
              tunnel: [w290 _] -> w284
              tunnel: w282 -> [w289 _]
              frame False {
                n145 = local read "Parameter Map Set"() -> (w286:u16)
                n146 = local read "Map Parameter"() -> (w285:u16)
                n147 = Bundle(cluster=T22 {"Parameter Map Set"=0, "Map Parameter"=0}, "Parameter Map Set"=w286, "Map Parameter"=w285) -> (w287:T22)
                n148 = Bundle By Name(cluster=w289, "Data"=w287) -> (w291:T7)
                n149 = Build Array(w291) -> (w290:T7[])
              }
              frame True {
              }
            }
          }
        }
        n150 = Unbundle By Name(w274) -> ("Parameter Map Display Range Event"=w277:refnum<event-registration>)
        n151 = register-events(reference=w277, w273, w272, w272, w272) -> (reference out=w276:refnum<event-registration>)  [unwired: 1 in, 1 out]
        n152 = Bundle By Name(cluster=w274, "Parameter Map Display Range Event"=w276) -> (w275:T5)
      }
      event User Event {
        n153 = event-data() -> ("subpanel"=w294:string, "event"=w293:string)  [unwired: 1 in]
        n154 = case shown="\"AlliGator\"" w294 {
          tunnel: w293 -> [_ w296]
          tunnel: [_ w295] -> w292
          frame "False", Default {
          }
          frame "AlliGator" {
            n155 = case shown="\"quit\"" w296 {
              tunnel: [_ TRUE] -> w295
              frame "False", Default {
              }
              frame "quit" {
              }
            }
          }
        }
      }
      event Panel Close? {
        w298 = TRUE ("Pin Button")
        n156 = event-data() -> ()  [unwired: 1 in, 1 out]
        n157 = property on="Pin Button" class="Bool (strict)"("Value"=w298) -> (error out=w301:errorcluster)  [unwired: 2 in, 1 out]
        n158 = call "AlliGator Dock-Undock Subpanel Event.vi"("Error In"=w301, "Dock?"=w298, "VI in"=w299) -> ("Error Out"=w300:errorcluster)  [unwired: 8 in]
        n159 = event-data("Discard?"=w298) -> ()  [unwired: 1 in, 1 out]
      }
    }
    n160 = call "AlliGator Settings Storage.vi"("AlliGator Settings List"=AlliGator_Settings_List."Miscellaneous:Verbose Error Mode") -> ("Variant Data out"=w57:variant)  [unwired: 9 in, 1 out]
    n161 = call-poly "Variant to Data.vi"("Variant"=w57) -> ("Value"=w50:bool)  [unwired: 8 in]
    n162 = call "Send Message to Notebook.vi"("Error In"=w52, "Text"=w49, "Notebook Queue"=w51) -> ("Error Out"=w54:errorcluster, "Notebook Queue"=w53:refnum<queue>)  [unwired: 5 in]
    n163 = call "Light Theme Message Style.vi"() -> ()  [unwired: 1 out]
    n164 = call "AlliGator Queue Non Empty Events.vi"("Actions"=w47, "AlliGator Q"=w48) -> ()  [unwired: 9 in, 1 out]
    n165 = call "Send Error to Notebook.vi"("error in (no error)"=w54, "Verbose Error Messages (T)"=w50, "State Machine Case Error Source"="Image Display Panel", "Notebook Q"=w53) -> ("Error Out"=w42:errorcluster)  [unwired: 7 in]
  }
  n166 = property on="Parameter ROI Color" class="ColBox"("Val(Sgnl)"="Parameter ROI Color") -> ()  [unwired: 2 in, 2 out]
  n167 = call "Tiny Clear Error.vi"("Error In"=w34) -> ("no Error Out"=w33:errorcluster)  [unwired: 8 in]
  n168 = Unregister For Events(event registration refnum=w35) -> (error out=w30:errorcluster)  [unwired: 1 in]
  n169 = invoke class="VI" method="FP.Close"(reference=w8, error in=w33) -> (error out=w31:errorcluster)  [unwired: 1 in, 2 out]
  n170 = Merge Errors(w31, w30) -> (w29:errorcluster)
  n171 = call "Tiny Clear Error.vi"("Error In"=w29) -> ()  [unwired: 8 in, 1 out]
